vi "Write and Read.vi"(6 "读取字节数":u32=9, 8 "错误输入（无错误）":errorcluster, 10 "Command":string, 11 "VISA输入":refnum<visa-resource-name>) -> (0 "错误输出":errorcluster, 2 "read buffer":string, 3 "VISA输出":refnum<visa-resource-name>)   [LabVIEW 2026, in "UI-距离测量.lvlib"]
uses:
  c435f975-a0c2-4a78-9012-8a3faee0265a.vi
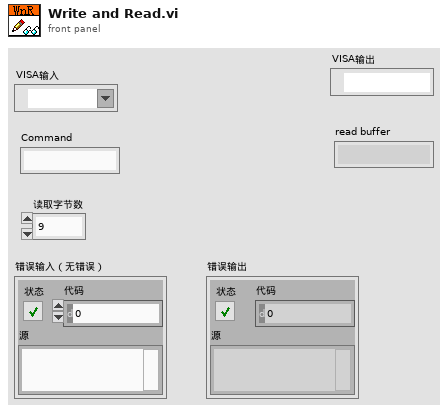
[diagram p1: front panel]
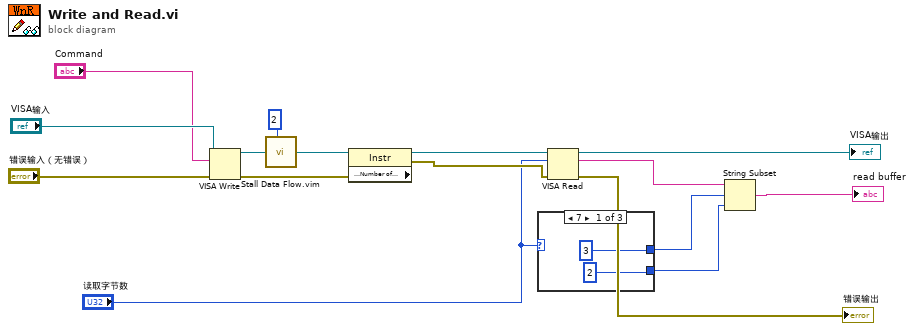
[diagram p0: block diagram]
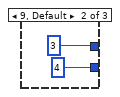
[diagram p2: hidden frame]
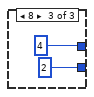
[diagram p3: hidden frame]
diagram:
  n1 = VISA Write(VISA resource name="VISA输入", write buffer="Command", error in (no error)="错误输入（无错误）") -> (VISA resource name out=w12:refnum<visa-resource-name>, error out=w14:errorcluster)  [unwired: 1 out]
  n2 = call "Stall Data Flow.vim"("value in"=w12, "milliseconds to wait"=u32 2) -> ("value out"=w13:refnum<visa-resource-name>)  [unwired: 1 out]
  n3 = property class="Instr" props=["Serial Settings:Number of Bytes at Serial Port"](reference=w13, error in=w14) -> (reference out=w6:refnum<visa-resource-name>, error out=w7:errorcluster)  [unwired: 1 out]
  n4 = case shown="7" "读取字节数" {
    tunnel: [3 ("偏移量(0)") 3 ("偏移量(0)") 4 ("偏移量(0)")] -> w4
    tunnel: [2 ("长度（剩余）") 4 ("长度（剩余）") 2 ("长度（剩余）")] -> w3
    frame 7 {
    }
    frame 9, Default {
    }
    frame 8 {
    }
  }
  n5 = VISA Read(VISA resource name=w6, byte count="读取字节数", error in (no error)=w7) -> (VISA resource name out=→"VISA输出":refnum<visa-resource-name>, read buffer=w11:string, error out=→"错误输出":errorcluster)  [unwired: 1 out]
  n6 = String Subset(string=w11, offset (0)=w4, length (rest)=w3) -> (substring=→"read buffer":string)
